vi "RFH-convert-water_calib_file.vi"() -> ()   [LabVIEW 2020, in "RFH-Reflection_File_Handler.lvlib"]
doc: "Run by hand: converts a water reference file to a water calibration file on the frequencies of a LibreVNA file and verifies it. The user picks the files, the save path and name, and the water temperature."
uses:
  RFH-Reflection_File_Handler.lvlib
  RFH-common_data_format.ctl
panel:
  out "Org Low Freq":dbl
  out "Org High Freq":dbl
  out "Converted High Freq":dbl
  out "Converted Low Freq":dbl
  out "Compare":T1(graph)
  out "All Good?":bool
  in  "Max Frequency (6G)":dbl=6000000000.0
  in  "Min Frequency  (0.3G)":dbl=300000000.0
  out "error out":errorcluster
  in  "Water temp C":dbl=25.0
  in  "Save Name":string
  in  "Save Path":path
  in  "LibreVNA samplerate file":path
  in  "Water filepath":path
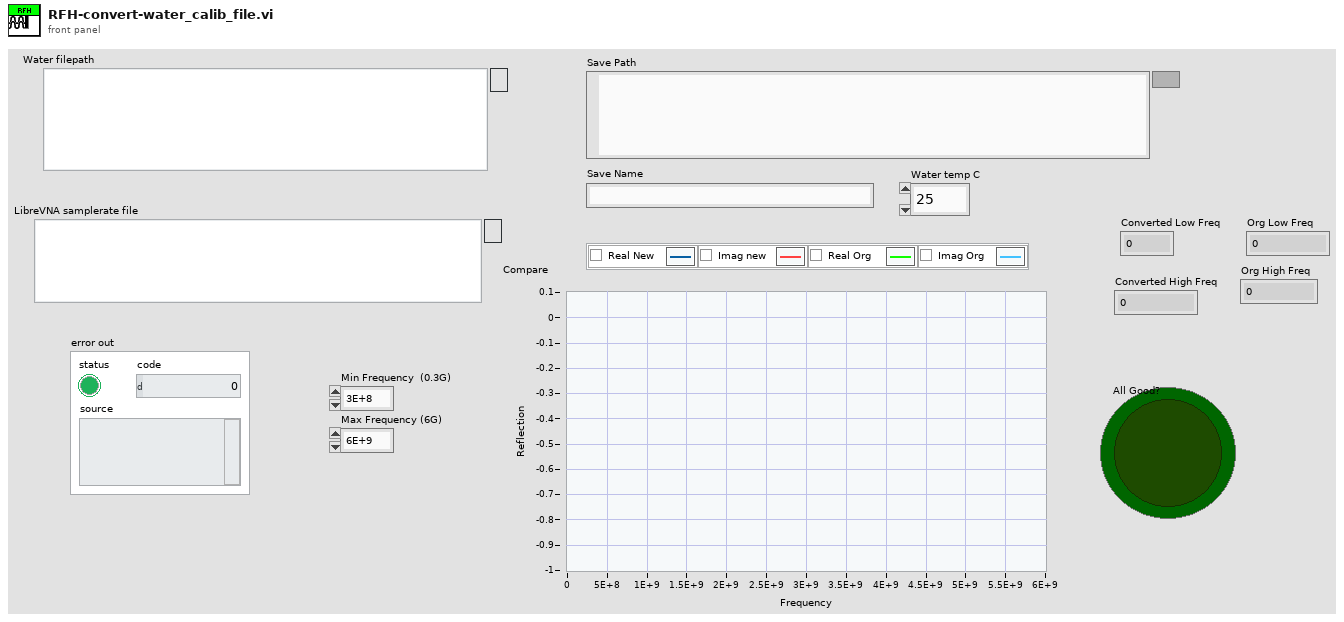
[diagram p1: front panel]
types:
  T1 = cluster{"Frequency":dbl[], "Reflection''":dbl[]}[]
  T2 = typedef "RFH-Reflection_File_Handler.lvlib/RFH-common_data_format.ctl" = cluster{"Frequency":dbl[], "Reflection'":dbl[], "Reflection''":dbl[], "Permativity'":dbl[], "Permativity''":dbl[], "Conductivity":dbl[], "Loss Tangent":dbl[], "Resistance":dbl[], "Reactance":dbl[]}
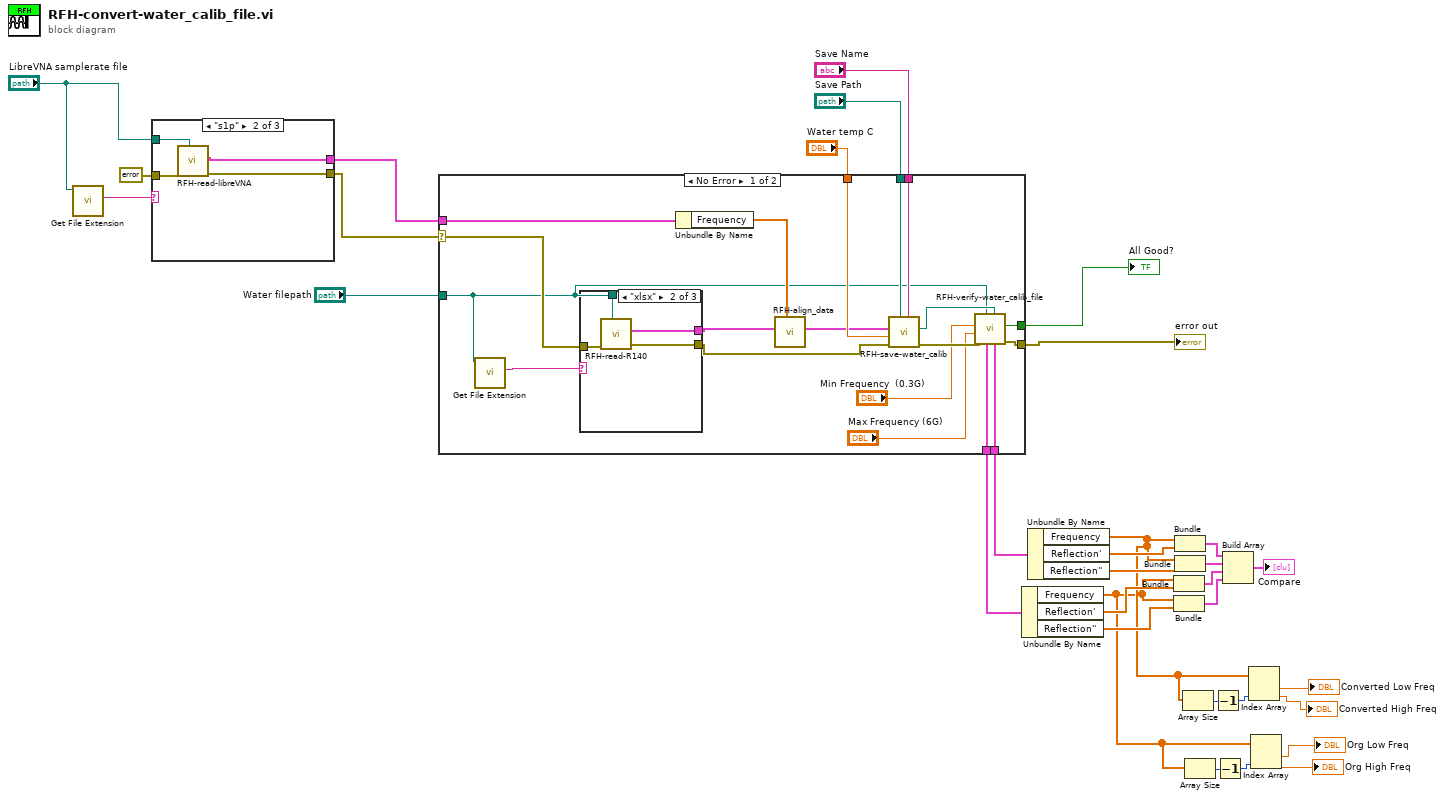
[diagram p0: block diagram]
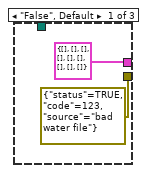
[diagram p2: hidden frame]
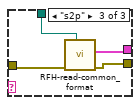
[diagram p3: hidden frame]
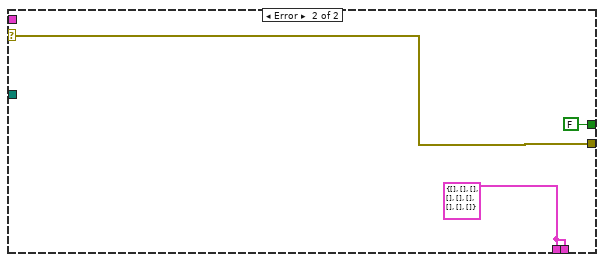
[diagram p4: hidden frame]
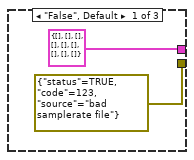
[diagram p5: hidden frame]
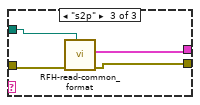
[diagram p6: hidden frame]
diagram:
  n1 = call <vilib>:"Get File Extension.vi"("file"="LibreVNA samplerate file") -> ("lowercase file extension"=w25:string)  [unwired: 6 in, 4 out]
  n2 = case shown="\"s1p\"" w25 {
    tunnel: [T2 {"Frequency"=[], "Reflection'"=[], "Reflection''"=[], "Permativity'"=[], "Permativity''"=[], "Conductivity"=[], "Loss Tangent"=[], "Resistance"=[], "Reactance"=[]} ("Common Format") w35 w41] -> w26
    tunnel: [errorcluster {"status"=TRUE, "code"=123, "source"="bad samplerate file"} ("error out") w36 w40] -> w27
    tunnel: errorcluster {"status"=FALSE, "code"=0, "source"=""} ("error out") -> [_ w37 w42]
    tunnel: "LibreVNA samplerate file" -> [_ w38 w39]
    frame "False", Default {
    }
    frame "s1p" {
      n3 = call "RFH-read-libreVNA.vi"("file path (dialog if empty)"=w38, "error in"=w37) -> ("error out"=w36:errorcluster, "Common Format"=w35:T2)  [unwired: 8 in]
    }
    frame "s2p" {
      n4 = call "RFH-read-common_format.vi"("file path (dialog if empty)"=w39, "error in"=w42) -> ("error out"=w40:errorcluster, "Common Format"=w41:T2)  [unwired: 8 in]
    }
  }
  n5 = case shown="No Error" w27 {
    selector: w27 -> [w54 w74]
    tunnel: w26 -> [w60 _]
    tunnel: "Save Path" -> [w58 _]
    tunnel: "Save Name" -> [w57 _]
    tunnel: "Water temp C" -> [w56 _]
    tunnel: [w51 w74] -> w23
    tunnel: "Water filepath" -> [w47 _]
    tunnel: [w46 FALSE ("All Good?")] -> w22
    tunnel: [w44 w72] -> w14
    tunnel: [w43 w72] -> w13
    frame No Error {
      n6 = call <vilib>:"Get File Extension.vi"("file"=w47) -> ("lowercase file extension"=w53:string)  [unwired: 6 in, 4 out]
      n7 = case shown="\"xlsx\"" w53 {
        tunnel: [T2 {"Frequency"=[], "Reflection'"=[], "Reflection''"=[], "Permativity'"=[], "Permativity''"=[], "Conductivity"=[], "Loss Tangent"=[], "Resistance"=[], "Reactance"=[]} ("Common Format") w67 w69] -> w61
        tunnel: w47 -> [_ w66 w70]
        tunnel: [errorcluster {"status"=TRUE, "code"=123, "source"="bad water file"} ("error out") w65 w68] -> w55
        tunnel: w54 -> [_ w64 w71]
        frame "False", Default {
        }
        frame "xlsx" {
          n8 = call "RFH-read-R140.vi"("file path (dialog if empty)"=w66, "error in (no error)"=w64) -> ("error out"=w65:errorcluster, "Common Format"=w67:T2)  [unwired: 7 in, 1 out]
        }
        frame "s2p" {
          n9 = call "RFH-read-common_format.vi"("file path (dialog if empty)"=w70, "error in"=w71) -> ("error out"=w68:errorcluster, "Common Format"=w69:T2)  [unwired: 8 in]
        }
      }
      n10 = Unbundle By Name(w60) -> ("Frequency"=w59:dbl[])
      n11 = call "RFH-align_data.vi"("Xi"=w59, "Common Format"=w61) -> ("Common Format alligned"=w45:T2)  [unwired: 9 in]
      n12 = call "RFH-save-water_calib.vi"("Save Name"=w57, "Save Path"=w58, "error in (no error)"=w55, "Water temp"=w56, "Common Format"=w45) -> ("error out"=w52:errorcluster, "Filepath"=w48:path)  [unwired: 5 in]
      n13 = call "RFH-verify-water_calib_file.vi"("Converted File"=w48, "Water filepath"=w47, "error in (no error)"=w52, "Max Frequency (6G)"="Max Frequency (6G)", "Min Frequency  (0.3G)"="Min Frequency  (0.3G)") -> ("error out"=w51:errorcluster, "All Good?"=w46:bool, "Converted"=w44:T2, "Original"=w43:T2)  [unwired: 3 in]
    }
    frame Error {
      w72 = T2 {"Frequency"=[], "Reflection'"=[], "Reflection''"=[], "Permativity'"=[], "Permativity''"=[], "Conductivity"=[], "Loss Tangent"=[], "Resistance"=[], "Reactance"=[]} ("Original")
    }
  }
  "error out" <- w23
  "All Good?" <- w22
  n14 = Unbundle By Name(w13) -> ("Frequency"=w5:dbl[], "Reflection'"=w16:dbl[], "Reflection''"=w15:dbl[])
  n15 = Unbundle By Name(w14) -> ("Frequency"=w8:dbl[], "Reflection'"=w21:dbl[], "Reflection''"=w20:dbl[])
  n16 = Bundle("Frequency"=w5, "Reflection'"=w16) -> (w12:cluster{"Frequency":dbl[], "Reflection'":dbl[]})  [unwired: 1 in]
  n17 = Bundle("Frequency"=w5, "Reflection''"=w15) -> (w11:cluster{"Frequency":dbl[], "Reflection''":dbl[]})  [unwired: 1 in]
  n18 = Bundle("Frequency"=w8, "Reflection'"=w21) -> (w19:cluster{"Frequency":dbl[], "Reflection'":dbl[]})  [unwired: 1 in]
  n19 = Bundle("Frequency"=w8, "Reflection''"=w20) -> (w18:cluster{"Frequency":dbl[], "Reflection''":dbl[]})  [unwired: 1 in]
  n20 = Array Size(array=w8) -> (size(s)=w9:i32)
  n21 = Array Size(array=w5) -> (size(s)=w7:i32)
  n22 = Decrement(x=w9) -> (x-1=w10:i32)
  n23 = Decrement(x=w7) -> (x-1=w6:i32)
  n24 = Build Array(w19, w18, w12, w11) -> (→"Compare":T1)
  n25 = Index Array(array=w8, index #2=w10) -> (element #1=→"Converted Low Freq":dbl, element #2=→"Converted High Freq":dbl)  [unwired: 1 in]
  n26 = Index Array(array=w5, index #2=w6) -> (element #1=→"Org Low Freq":dbl, element #2=→"Org High Freq":dbl)  [unwired: 1 in]
